vi "Sequence.CreateStepLoop.vi"(7 "Iteration":string, 8 "error in (no error)":errorcluster, 10 "Duration":dbl, 11 "Elements":T1[](array[typedef])) -> (0 "error out":errorcluster, 3 "Tasks":refnum<k24>[](array[refnum]))   [LabVIEW 2015, in "Simple Sequence Tools - Editor.lvlib"]
uses:
  Simple Sequence Tools - Editor.lvlib
  NationalInstruments.VeriStand.RealTimeSequenceDefinitionApi
  Types/Compiled.StepElementProperties.ctl
  Shared/Types/Channel.Properties.ctl
  Shared/Types/Step.Types.ctl
  Shared/SubVIs/Main.Constants.vi
  Shared/Simple Sequence Tools - Shared.lvlib
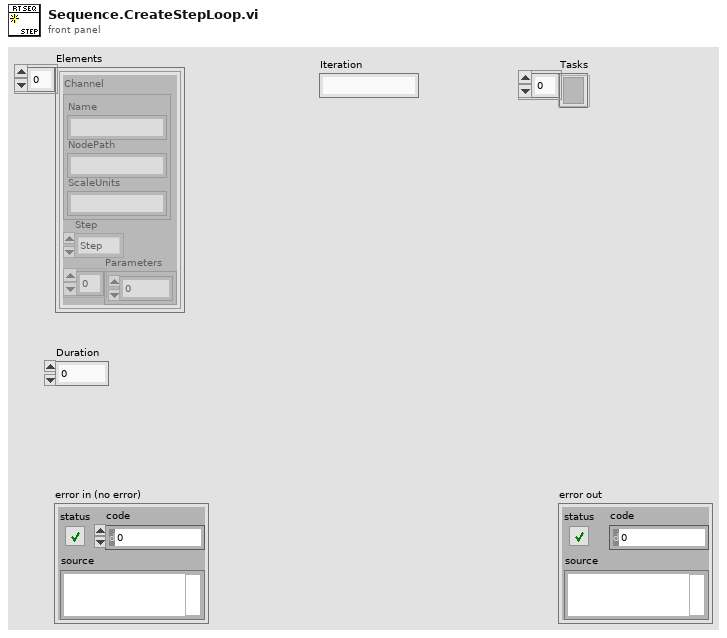
[diagram p1: front panel]
types:
  T1 = typedef "Simple Sequence Tools - Editor.lvlib/Compiled.StepElementProperties.ctl" = cluster{"Channel":T2, "Step":T3, "Parameters":dbl[]}
  T2 = typedef "Simple Sequence Tools - Shared.lvlib/Channel.Properties.ctl" = cluster{"Name":string, "NodePath":string, "ScaleUnits":string}
  T3 = typedef "Simple Sequence Tools - Shared.lvlib/Step.Types.ctl" = enum8{"Step", "iStep", "Ramp", "Unchanged", "Unknown", "Sine", "LogSine", "LinearSine", "ForcedRamp", "SquareWave"}
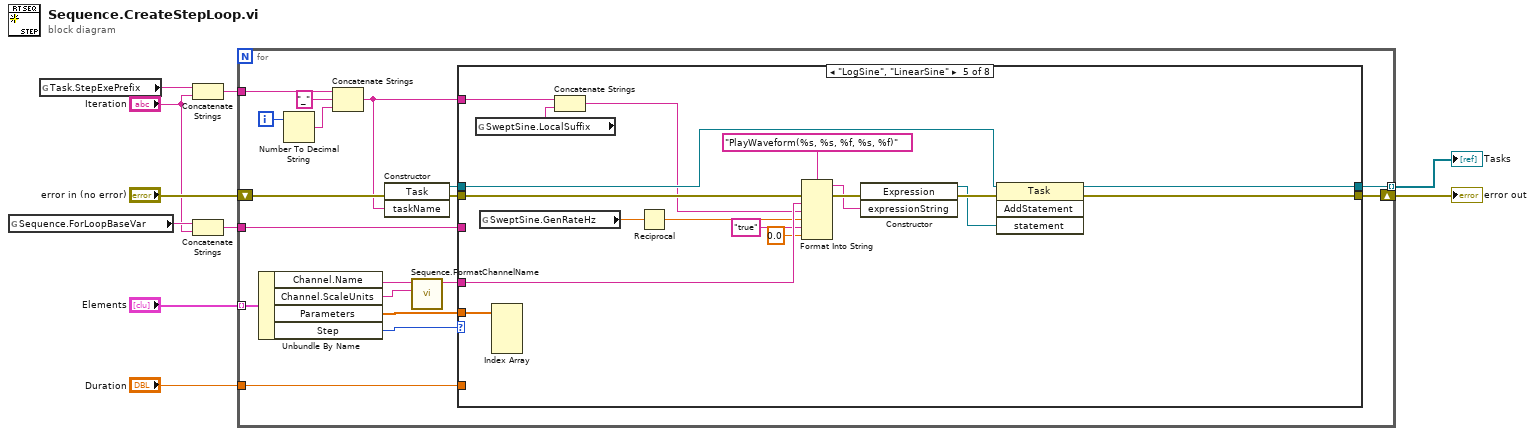
[diagram p0: block diagram]
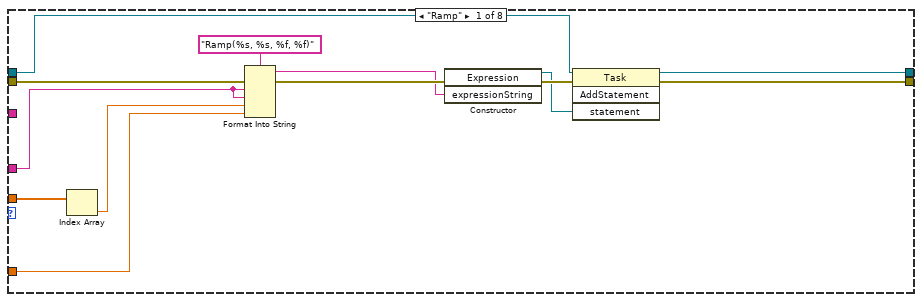
[diagram p2: hidden frame]
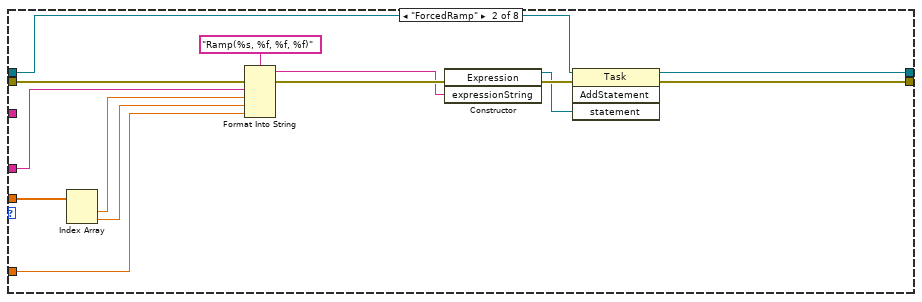
[diagram p3: hidden frame]
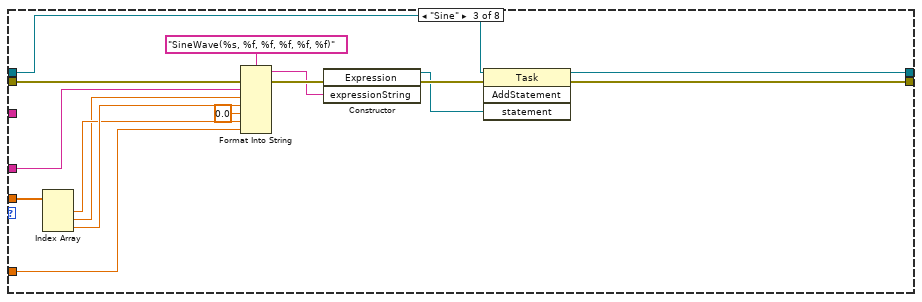
[diagram p4: hidden frame]
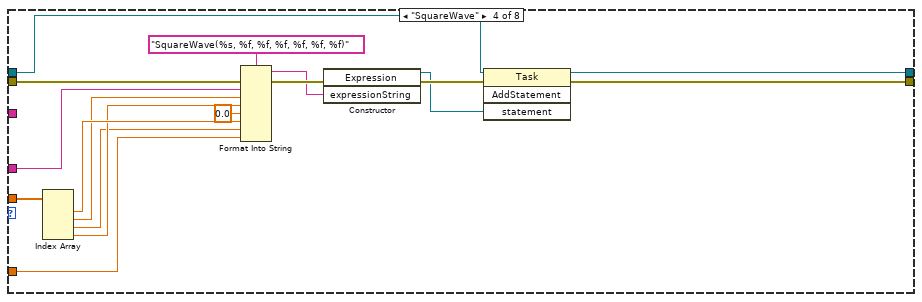
[diagram p5: hidden frame]
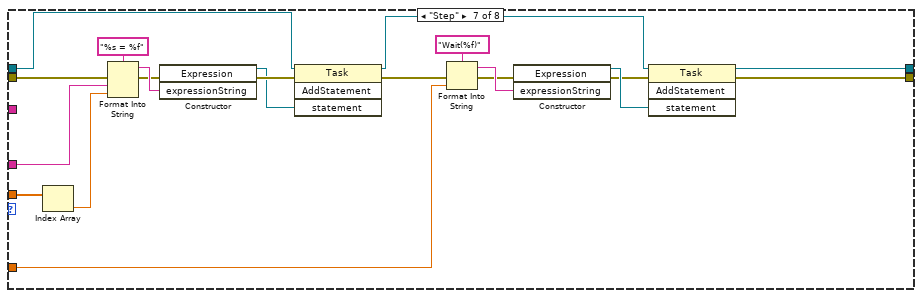
[diagram p7: hidden frame]
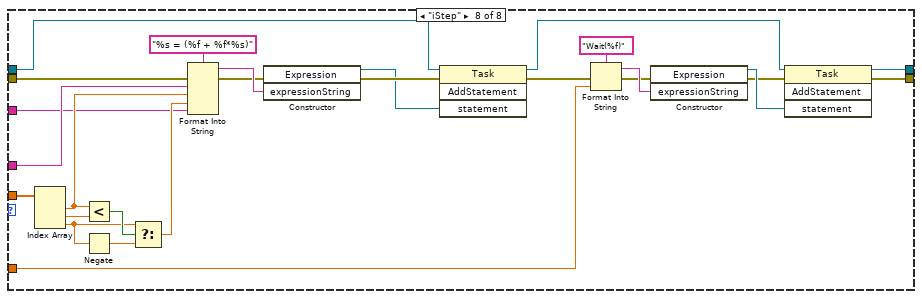
[diagram p8: hidden frame]
diagram:
  n1 = global read "Main.Constants.vi" "Sequence.ForLoopBaseVar"() -> (w3:string)
  n2 = global read "Main.Constants.vi" "Task.StepExePrefix"() -> (w5:string)
  n3 = Concatenate Strings(w5, "Iteration") -> (w4:string)
  n4 = Concatenate Strings(w3, "Iteration") -> (w1:string)
  n5 = for {
    tunnel: "Elements" -> [w24] mode=indexing
    shift-right: [w15] -> w9
    shift-left: "error in (no error)" -> [w23]
    tunnel: w4 -> [w27]
    tunnel: [w13] -> w10 mode=indexing
    tunnel: "Duration" -> [w19]
    tunnel: w1 -> [w12]
    i -> [w28]
    n6 = Unbundle By Name(w24) -> ("Channel.Name"=w22:string, "Channel.ScaleUnits"=w21:string, "Parameters"=w18:dbl[], "Step"=w17:T3)
    n7 = Number To Decimal String(number=w28) -> (decimal integer string=w25:string)  [unwired: 1 in]
    n8 = Concatenate Strings(w27, "_" ("string"), w25) -> (w11:string)
    n9 = constructor class="Task"(error in=w23, "taskName"=w11) -> (reference out=w14:refnum<k24>, error out=w16:errorcluster)  [unwired: 2 in, 2 out]
    n10 = call "Sequence.FormatChannelName.vi"("ScaleUnits"=w21, "Name"=w22) -> ("ChannelName"=w20:string)  [unwired: 9 in]
    n11 = case shown="\"LogSine\", \"LinearSine\"" w17 {
      tunnel: w20 -> [w41 w55 w70 w87 w105 _ w127 w153]
      tunnel: w18 -> [w30 w43 w69 w86 w104 _ w126 w152]
      tunnel: w19 -> [w39 w52 w58 w76 _ _ w117 w144]
      tunnel: [w33 w46 w63 w80 w98 w107 w111 w138] -> w15
      tunnel: w16 -> [w38 w51 w68 w85 w103 w107 w124 w151]
      tunnel: w14 -> [w35 w48 w65 w82 w100 w108 w116 w143]
      tunnel: [w32 w45 w62 w79 w97 w108 w109 w136] -> w13
      tunnel: w12 -> [_ _ _ _ _ _ _ w129]
      tunnel: w11 -> [_ _ _ _ w92 _ _ _]
      frame "Ramp" {
        n12 = Index Array(array=w30) -> (element=w40:dbl)  [unwired: 1 in]
        n13 = Format Into String(format string="Ramp(%s, %s, %f, %f)" ("expressionString"), error in=w38, w41, w41, w40, w39) -> (resulting string=w31:string, error out=w34:errorcluster)  [unwired: 1 in]
        n14 = constructor class="Expression"(error in=w34, "expressionString"=w31) -> (reference out=w36:refnum<k24>, error out=w37:errorcluster)  [unwired: 2 in, 2 out]
        n15 = invoke class="Task" method="AddStatement"(reference=w35, error in=w37, "statement"=w36) -> (reference out=w32:refnum<k24>, error out=w33:errorcluster)  [unwired: 1 in, 2 out]
      }
      frame "ForcedRamp" {
        n16 = Index Array(array=w43) -> (element #1=w54:dbl, element #2=w53:dbl)  [unwired: 2 in]
        n17 = Format Into String(format string="Ramp(%s, %f, %f, %f)" ("expressionString"), error in=w51, w55, w54, w53, w52) -> (resulting string=w44:string, error out=w47:errorcluster)  [unwired: 1 in]
        n18 = constructor class="Expression"(error in=w47, "expressionString"=w44) -> (reference out=w49:refnum<k24>, error out=w50:errorcluster)  [unwired: 2 in, 2 out]
        n19 = invoke class="Task" method="AddStatement"(reference=w48, error in=w50, "statement"=w49) -> (reference out=w45:refnum<k24>, error out=w46:errorcluster)  [unwired: 1 in, 2 out]
      }
      frame "Sine" {
        n20 = Index Array(array=w69) -> (element #1=w57:dbl, element #2=w56:dbl, element #3=w60:dbl)  [unwired: 3 in]
        n21 = Format Into String(format string="SineWave(%s, %f, %f, %f, %f, %f)" ("expressionString"), error in=w68, w70, w56, w60, 0.0 ("input 4"), w57, w58) -> (resulting string=w61:string, error out=w64:errorcluster)  [unwired: 1 in]
        n22 = constructor class="Expression"(error in=w64, "expressionString"=w61) -> (reference out=w66:refnum<k24>, error out=w67:errorcluster)  [unwired: 2 in, 2 out]
        n23 = invoke class="Task" method="AddStatement"(reference=w65, error in=w67, "statement"=w66) -> (reference out=w62:refnum<k24>, error out=w63:errorcluster)  [unwired: 1 in, 2 out]
      }
      frame "SquareWave" {
        n24 = Index Array(array=w86) -> (element #1=w75:dbl, element #2=w74:dbl, element #3=w72:dbl, element #4=w73:dbl)  [unwired: 4 in]
        n25 = Format Into String(format string="SquareWave(%s, %f, %f, %f, %f, %f, %f)" ("expressionString"), error in=w85, w87, w74, w73, 0.0 ("input 4"), w75, w72, w76) -> (resulting string=w78:string, error out=w81:errorcluster)  [unwired: 1 in]
        n26 = constructor class="Expression"(error in=w81, "expressionString"=w78) -> (reference out=w83:refnum<k24>, error out=w84:errorcluster)  [unwired: 2 in, 2 out]
        n27 = invoke class="Task" method="AddStatement"(reference=w82, error in=w84, "statement"=w83) -> (reference out=w79:refnum<k24>, error out=w80:errorcluster)  [unwired: 1 in, 2 out]
      }
      frame "LogSine", "LinearSine" {
        n28 = global read "Main.Constants.vi" "SweptSine.LocalSuffix"() -> (w90:string)
        n29 = global read "Main.Constants.vi" "SweptSine.GenRateHz"() -> (w89:dbl)
        n30 = Index Array(array=w104) -> ()  [unwired: 4 in, 4 out]
        n31 = Concatenate Strings(w92, w90) -> (w91:string)
        n32 = Reciprocal(x=w89) -> (1/x=w93:dbl)
        n33 = Format Into String(format string="PlayWaveform(%s, %s, %f, %s, %f)" ("expressionString"), error in=w103, w105, w91, w93, "true" ("input 4"), 0.0 ("input 4")) -> (resulting string=w96:string, error out=w99:errorcluster)  [unwired: 1 in]
        n34 = constructor class="Expression"(error in=w99, "expressionString"=w96) -> (reference out=w101:refnum<k24>, error out=w102:errorcluster)  [unwired: 2 in, 2 out]
        n35 = invoke class="Task" method="AddStatement"(reference=w100, error in=w102, "statement"=w101) -> (reference out=w97:refnum<k24>, error out=w98:errorcluster)  [unwired: 1 in, 2 out]
      }
      frame "Unchanged", Default {
      }
      frame "Step" {
        n36 = Index Array(array=w126) -> (element=w125:dbl)  [unwired: 1 in]
        n37 = Format Into String(format string="%s = %f" ("expressionString"), error in=w124, w127, w125) -> (resulting string=w121:string, error out=w112:errorcluster)  [unwired: 1 in]
        n38 = constructor class="Expression"(error in=w112, "expressionString"=w121) -> (reference out=w122:refnum<k24>, error out=w123:errorcluster)  [unwired: 2 in, 2 out]
        n39 = invoke class="Task" method="AddStatement"(reference=w116, error in=w123, "statement"=w122) -> (reference out=w110:refnum<k24>, error out=w113:errorcluster)  [unwired: 1 in, 2 out]
        n40 = Format Into String(format string="Wait(%f)", error in=w113, w117) -> (resulting string=w115:string, error out=w114:errorcluster)  [unwired: 1 in]
        n41 = constructor class="Expression"(error in=w114, "expressionString"=w115) -> (reference out=w120:refnum<k24>, error out=w119:errorcluster)  [unwired: 2 in, 2 out]
        n42 = invoke class="Task" method="AddStatement"(reference=w110, error in=w119, "statement"=w120) -> (reference out=w109:refnum<k24>, error out=w111:errorcluster)  [unwired: 1 in, 2 out]
      }
      frame "iStep" {
        n43 = Index Array(array=w152) -> (element #1=w135:dbl, element #2=w134:dbl, element #3=w131:dbl)  [unwired: 3 in]
        n44 = Less?(x=w135, y=w134) -> (x < y?=w133:bool)
        n45 = Negate(x=w131) -> (-x=w132:dbl)
        n46 = Select(t=w131, s=w133, f=w132) -> (s? t:f=w130:dbl)
        n47 = Format Into String(format string="%s = (%f + %f*%s)" ("expressionString"), error in=w151, w153, w135, w130, w129) -> (resulting string=w148:string, error out=w139:errorcluster)  [unwired: 1 in]
        n48 = constructor class="Expression"(error in=w139, "expressionString"=w148) -> (reference out=w149:refnum<k24>, error out=w150:errorcluster)  [unwired: 2 in, 2 out]
        n49 = invoke class="Task" method="AddStatement"(reference=w143, error in=w150, "statement"=w149) -> (reference out=w137:refnum<k24>, error out=w140:errorcluster)  [unwired: 1 in, 2 out]
        n50 = Format Into String(format string="Wait(%f)", error in=w140, w144) -> (resulting string=w142:string, error out=w141:errorcluster)  [unwired: 1 in]
        n51 = constructor class="Expression"(error in=w141, "expressionString"=w142) -> (reference out=w147:refnum<k24>, error out=w146:errorcluster)  [unwired: 2 in, 2 out]
        n52 = invoke class="Task" method="AddStatement"(reference=w137, error in=w146, "statement"=w147) -> (reference out=w136:refnum<k24>, error out=w138:errorcluster)  [unwired: 1 in, 2 out]
      }
    }
  }
  "Tasks" <- w10
  "error out" <- w9
